vi "Discover Tests.vi"(8 "error in (no error)":errorcluster, 11 "Test Runner in":refnum<class "Test Runner.lvclass">) -> (0 "error out":errorcluster, 3 "Test Runner out":refnum<class "Test Runner.lvclass">)   [LabVIEW 2020, in "Caraya.lvlib" / "Test Runner.lvclass"]
uses:
  Test Runner.lvclass
  Test Runner.lvclass/Test Runner.ctl
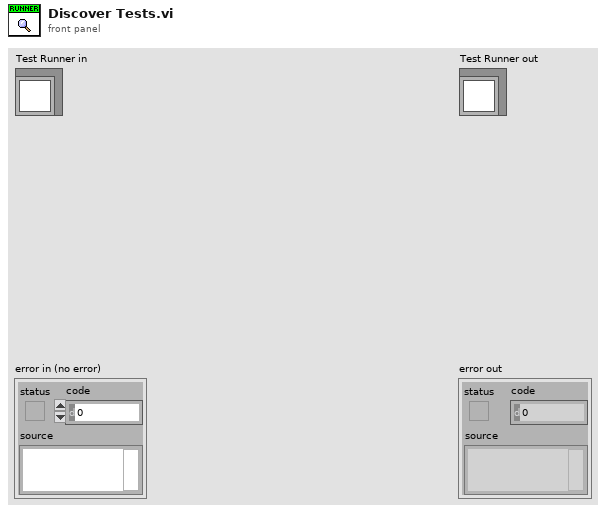
[diagram p1: front panel]
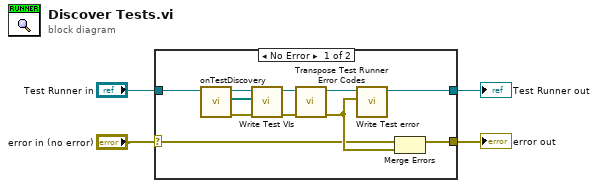
[diagram p0: block diagram]
diagram:
  n1 = case shown="No Error" "error in (no error)" {
    selector: "error in (no error)" -> [w7 w17]
    tunnel: [w14 w17] -> w4
    tunnel: "Test Runner in" -> [w15 w16]
    tunnel: [w5 w16] -> w2
    frame No Error {
      n2 = call-dynamic "onTestDiscovery.vi"("Test Runner in"=w15) -> ("error out"=w9:errorcluster, "Tests VIs"=w10:path[], "Test Runner out"=w11:refnum<class "Test Runner.lvclass">)  [unwired: 8 in]
      n3 = call "Write Test VIs.vi"("error in (no error)"=w9, "Test VIs"=w10, "Test Runner in"=w11) -> ("error out"=w8:errorcluster, "Test Runner out"=w6:refnum<class "Test Runner.lvclass">)  [unwired: 7 in]
      n4 = call-dynamic "Transpose Test Runner Error Codes.vi"("error in (no error)"=w8, "Test Runner in"=w6) -> ("error out"=w12:errorcluster, "Test Runner out"=w13:refnum<class "Test Runner.lvclass">)  [unwired: 8 in]
      n5 = call "Write Test error.vi"("Test error"=w12, "Test Runner in"=w13) -> ("Test Runner out"=w5:refnum<class "Test Runner.lvclass">)  [unwired: 9 in]
      n6 = Merge Errors(w7, w12) -> (w14:errorcluster)
    }
    frame Error {
    }
  }
  "error out" <- w4
  "Test Runner out" <- w2
